vi "Destroy User Events.vi"(11 "UI Template in":refnum<class "ChannelManagerUI.lvclass">) -> (3 "UI Template out":refnum<class "ChannelManagerUI.lvclass">)   [LabVIEW 2021, in "Channel.lvlib" / "ChannelManagerUI.lvlib" / "ChannelManagerUI.lvclass"]
uses:
  ChannelManagerUI.lvclass
  ChannelManagerUI.lvclass/ChannelManagerUI.ctl
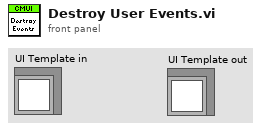
[diagram p1: front panel]
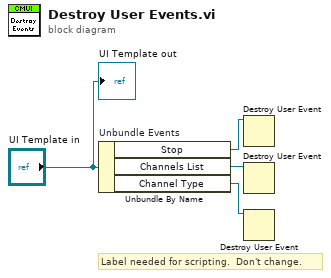
[diagram p0: block diagram]
diagram:
  # "Label needed for scripting.  Don't change."
  n1 = Unbundle By Name "Unbundle Events"("UI Template in") -> ("Stop"=w3:refnum<user-event>, "Channels List"=w2:refnum<user-event>, "Channel Type"=w1:refnum<user-event>)
  n2 = Destroy User Event(user event=w3) -> ()  [unwired: 1 in, 1 out]
  n3 = Destroy User Event(user event=w2) -> ()  [unwired: 1 in, 1 out]
  n4 = Destroy User Event(user event=w1) -> ()  [unwired: 1 in, 1 out]
  "UI Template out" <- "UI Template in"
